vi "Handle Incoming Packets.vi"(8 "error in (no error)":errorcluster, 9 "SessionMailbox":refnum<queue>, 10 "Incoming Packet":refnum<class "ControlPacket.lvclass">, 11 "Server in":refnum<class "Server.lvclass">) -> (0 "error out":errorcluster, 1 "SessionMailbox out":refnum<queue>, 2 "Outgoing":T1, 3 "Server out":refnum<class "Server.lvclass">)   [LabVIEW 2013, in "MQTT Server.lvlib" / "Server.lvclass"]
uses:
  Server.lvclass
  <vilib>/LabVIEW Open Source Project/MQTT Control Packets/Control Packets/ControlPacket/ControlPacket.lvclass
  <vilib>/LabVIEW Open Source Project/MQTT Connection/MQTT_Base/Base Class/Response -- cluster.ctl
  Server.lvclass/Server.ctl
  PacketTracer/PacketTracer.lvclass
  <vilib>/LabVIEW Open Source Project/MQTT Connection/MQTT_Base/Base Class/MQTT_Base.lvclass
  <vilib>/LabVIEW Open Source Project/MQTT Control Packets/Control Packets/CONNECT/CONNECT.lvclass
  <vilib>/LabVIEW Open Source Project/MQTT Control Packets/Control Packets/CONNACK/Connect Return Code -- enum.ctl
  <vilib>/LabVIEW Open Source Project/MQTT Control Packets/Control Packets/DISCONNECT/DISCONNECT.lvclass
  <vilib>/LabVIEW Open Source Project/MQTT Control Packets/Control Packets/PUBLISH/PUBLISH.lvclass
  <vilib>/LabVIEW Open Source Project/MQTT Connection/MQTT_Base/Base Class/MQTT_Base.lvclass/MQTT_Base.ctl
  <vilib>/LabVIEW Open Source Project/MQTT Control Packets/Control Packets/ControlPacket/ControlPacket.lvclass/ControlPacket.ctl
  <vilib>/LabVIEW Open Source Project/MQTT Control Packets/Control Packets/Ack/Ack.lvclass
  <vilib>/LabVIEW Open Source Project/MQTT Control Packets/Control Packets/PUBREL/PUBREL.lvclass
  <vilib>/LabVIEW Open Source Project/MQTT Control Packets/Control Packets/SUBSCRIBE/SUBSCRIBE.lvclass
  <vilib>/LabVIEW Open Source Project/MQTT Control Packets/Control Packets/SUBACK/Subscription Success Code.ctl
  <vilib>/LabVIEW Open Source Project/MQTT Control Packets/Control Packets/ControlPacket/QualityOfService -- enum.ctl
  <vilib>/LabVIEW Open Source Project/MQTT Control Packets/Control Packets/UNSUBSCRIBE/UNSUBSCRIBE.lvclass
  <vilib>/LabVIEW Open Source Project/MQTT Control Packets/Control Packets/PINGREQ/PINGREQ.lvclass
  PacketCollection/PacketCollection.lvclass/PacketCollection.ctl
  <vilib>/LabVIEW Open Source Project/MQTT Control Packets/Control Packets/PUBREC/PUBREC.lvclass
  <vilib>/LabVIEW Open Source Project/MQTT Control Packets/Control Packets/CONNACK/CONNACK.lvclass
  <vilib>/LabVIEW Open Source Project/MQTT Control Packets/Control Packets/SUBACK/SUBACK.lvclass
  PacketCollection/PacketCollection.lvclass
  <vilib>/LabVIEW Open Source Project/MQTT Control Packets/Control Packets/PINGRESP/PINGRESP.lvclass
  <vilib>/LabVIEW Open Source Project/MQTT Control Packets/Control Packets/UNSUBACK/UNSUBACK.lvclass
  StoredSessions/StoredSessions.lvclass
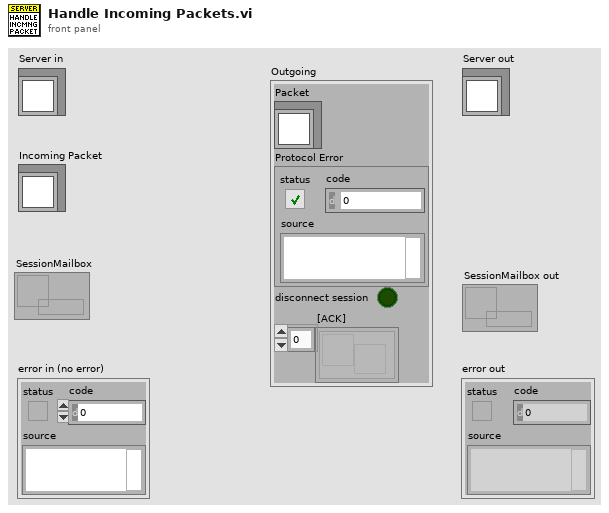
[diagram p1: front panel]
types:
  T1 = typedef "MQTT Base.lvlib/MQTT_Base.lvclass/Response -- cluster.ctl" = cluster{"Packet":refnum<class "ControlPacket.lvclass">, "Protocol Error":errorcluster, "disconnect session":bool, "[ACK]":refnum<notifier>[]}
  T2 = typedef "MQTT_Control_Packets.lvlib/CONNACK.lvclass/Connect Return Code -- enum.ctl" = enum16{"Connection accepted", "Unacceptable protocol version", "Identifier Rejected", "Server Unavailable", "Bad Username or Password", "Not Authorized"}
  T3 = typedef "MQTT_Control_Packets.lvlib/SUBACK.lvclass/Subscription Success Code.ctl" = cluster{"Subscription Failure":bool, "QoS":T4}
  T4 = typedef "MQTT_Control_Packets.lvlib/ControlPacket.lvclass/QualityOfService -- enum.ctl" = enum16{"0 (At Most Once)", "1 (At Least Once)", "2 (Exactly Once)"}
  T5 = typedef "MQTT_Control_Packets.lvlib/ControlPacket.lvclass/Control Packet Type -- enum.ctl" = enum16{"Reserved", "CONNECT", "CONNACK", "PUBLISH", "PUBACK", "PUBREC", "PUBREL", "PUBCOMP", "SUBSCRIBE", "SUBACK", "UNSUBSCRIBE", "UNSUBACK", "PINGREQ", "PINGRESP", "DISCONNECT", "AUTH"}
  T6 = typedef "MQTT_Control_Packets.lvlib/CONNECT.lvclass/ConnectPayload -- cluster.ctl" = cluster{"Will Topic":string, "Will Message":string, "Username":string, "Password":string}
  T7 = typedef "MQTT_Control_Packets.lvlib/CONNECT.lvclass/ConnectFlags -- cluster.ctl" = cluster{"Reserved":bool, "Clean Session":bool, "Will Flag":bool, "Will QoS 1":bool, "Will QoS 2":bool, "Will Retain":bool, "Password Flag":bool, "User Name Flag":bool}
  T8 = typedef "MQTT Server.lvlib/StoredSessions.lvclass/Session State -- cluster.ctl" = cluster{"Client ID":string, "Subscriptions":T9[], "PUBREC":u16[]}
  T9 = typedef "MQTT_Control_Packets.lvlib/SUBSCRIBE.lvclass/Topic Subscription -- cluster.ctl" = cluster{"Topic Filter":string, "QoS":T4}
  T10 = typedef "MQTT Base.lvlib/MQTT_Base.lvclass/Public Events -- cluster.ctl" = cluster{"Stop Event":refnum<user-event>, "Error Event":refnum<user-event>, "Inbound Message":refnum<user-event>}
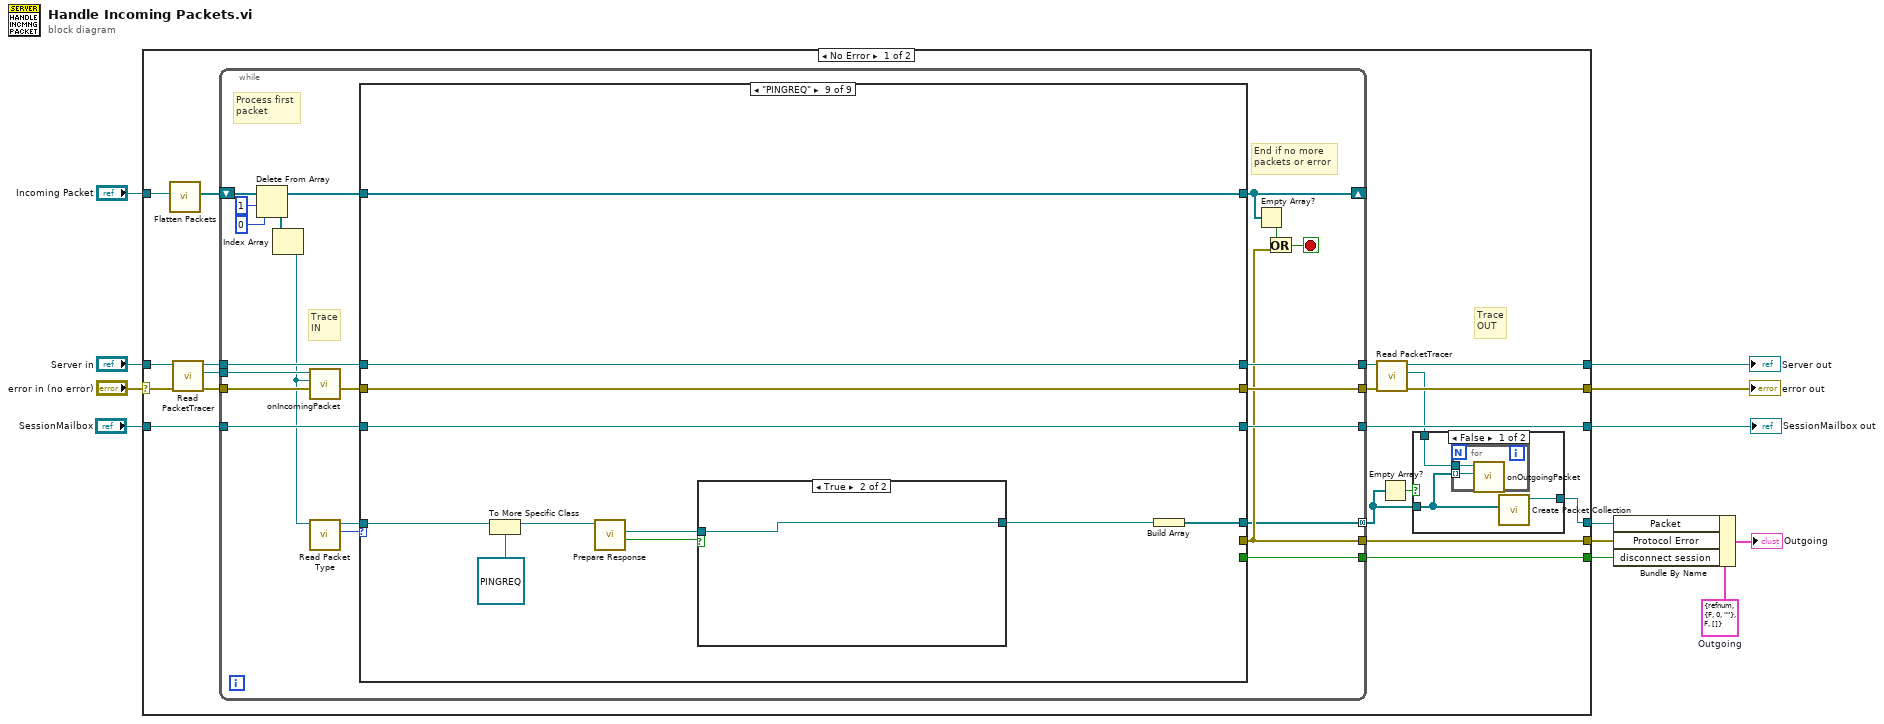
[diagram p0: block diagram]
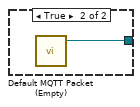
[diagram p2: hidden frame]
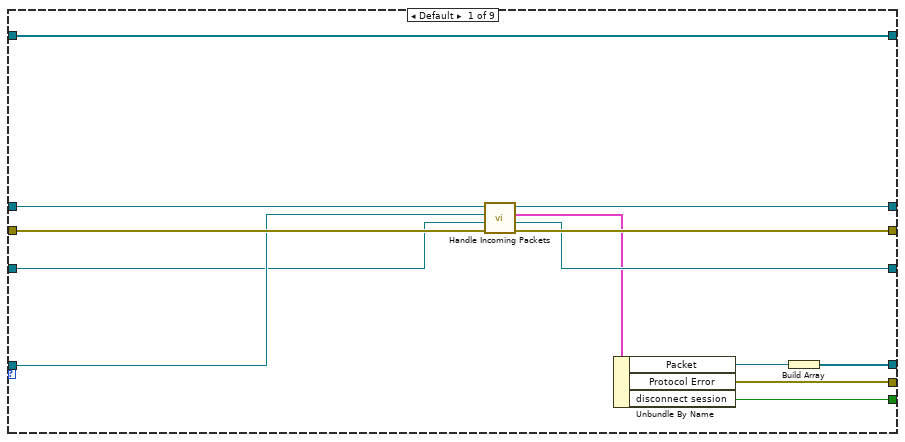
[diagram p3: hidden frame]
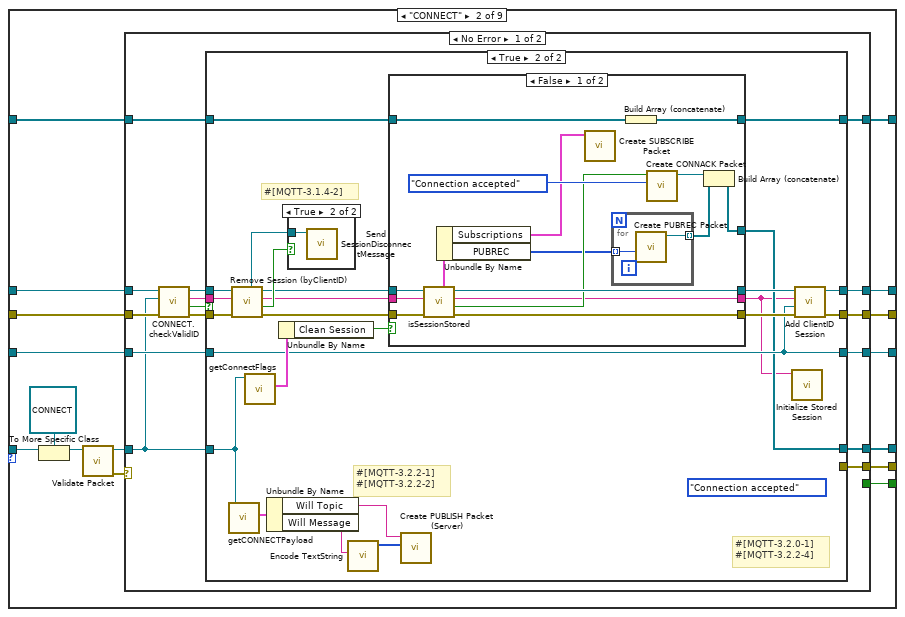
[diagram p4: hidden frame]
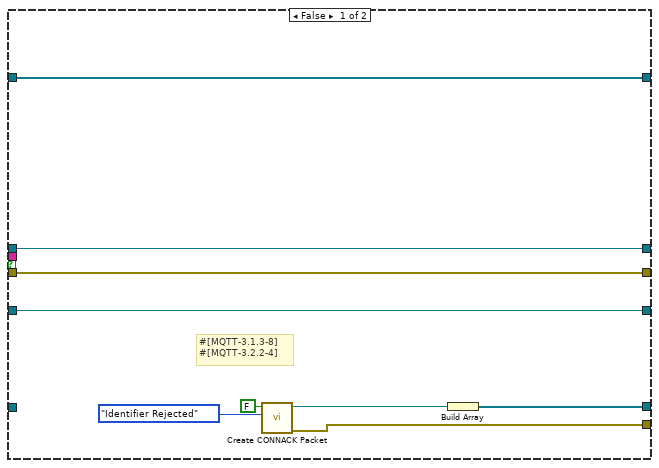
[diagram p5: hidden frame]
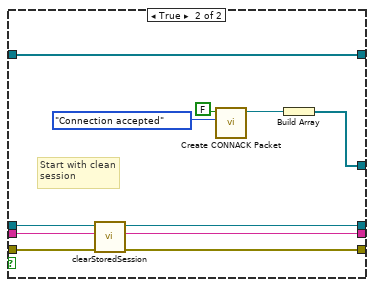
[diagram p6: hidden frame]
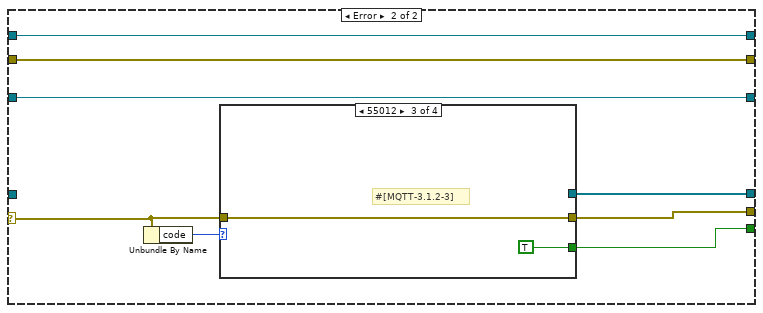
[diagram p8: hidden frame]
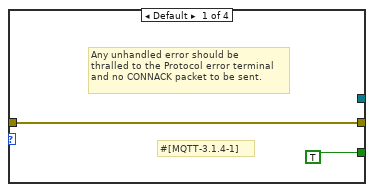
[diagram p9: hidden frame]
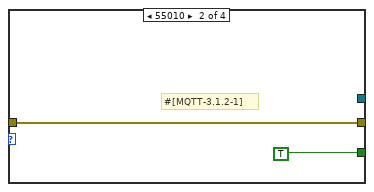
[diagram p10: hidden frame]
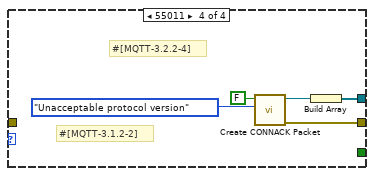
[diagram p11: hidden frame]
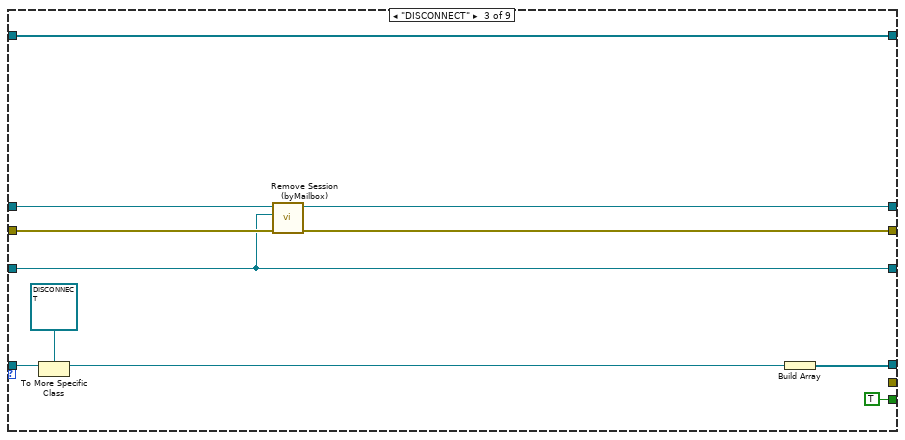
[diagram p12: hidden frame]
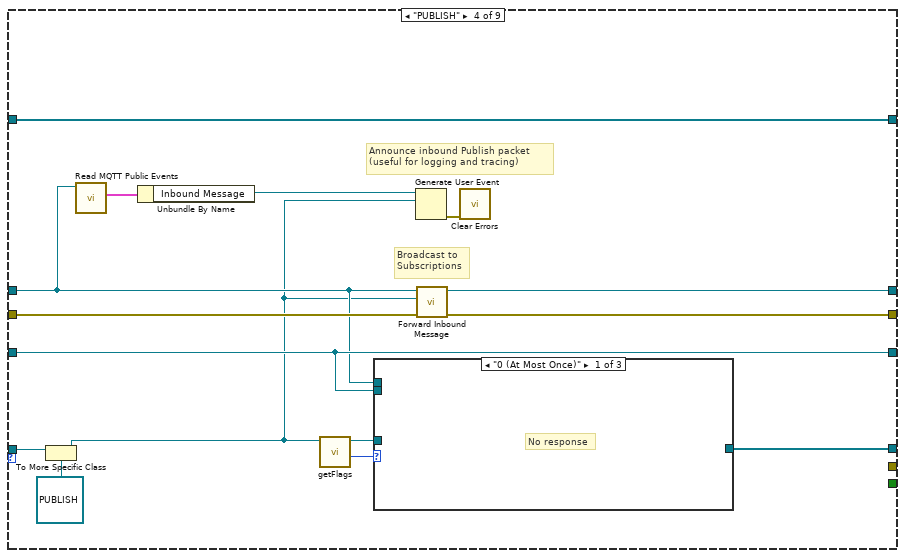
[diagram p13: hidden frame]
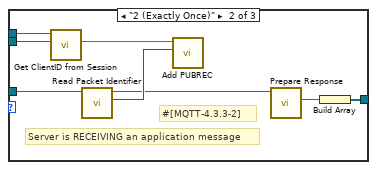
[diagram p14: hidden frame]
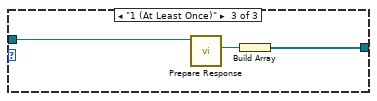
[diagram p15: hidden frame]
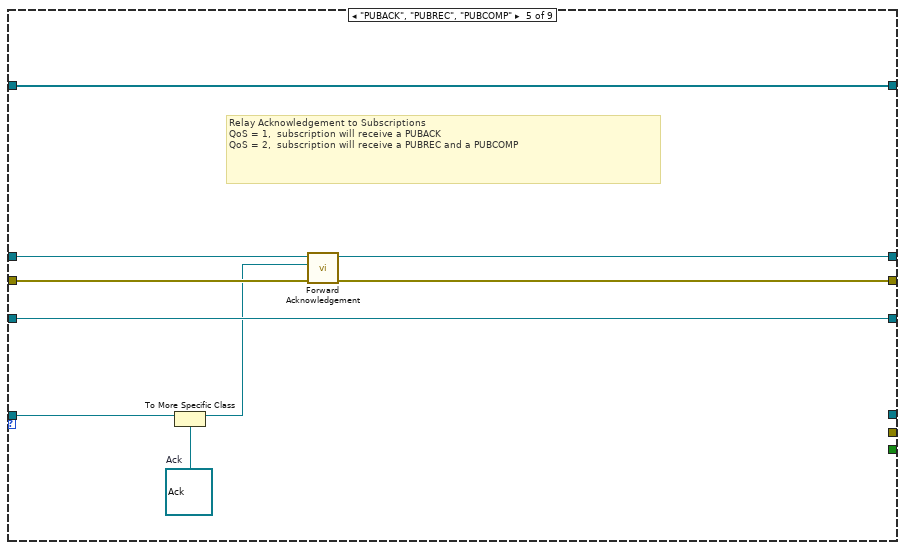
[diagram p16: hidden frame]
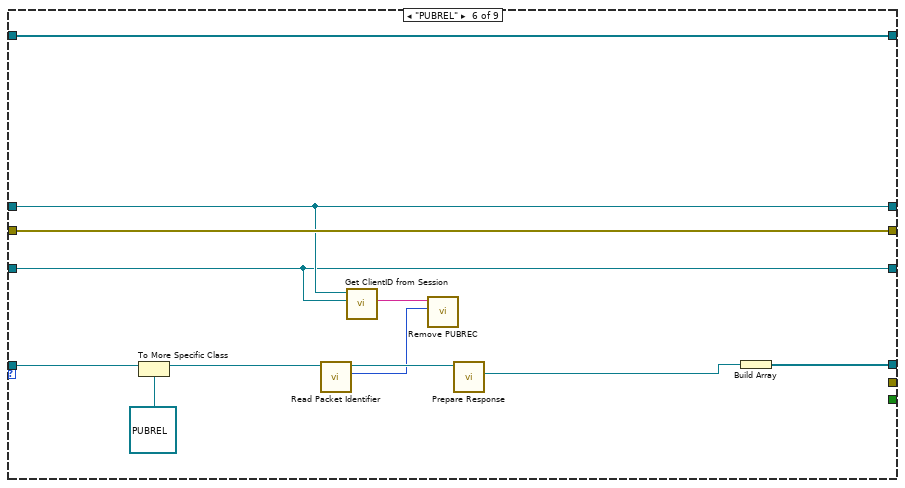
[diagram p17: hidden frame]
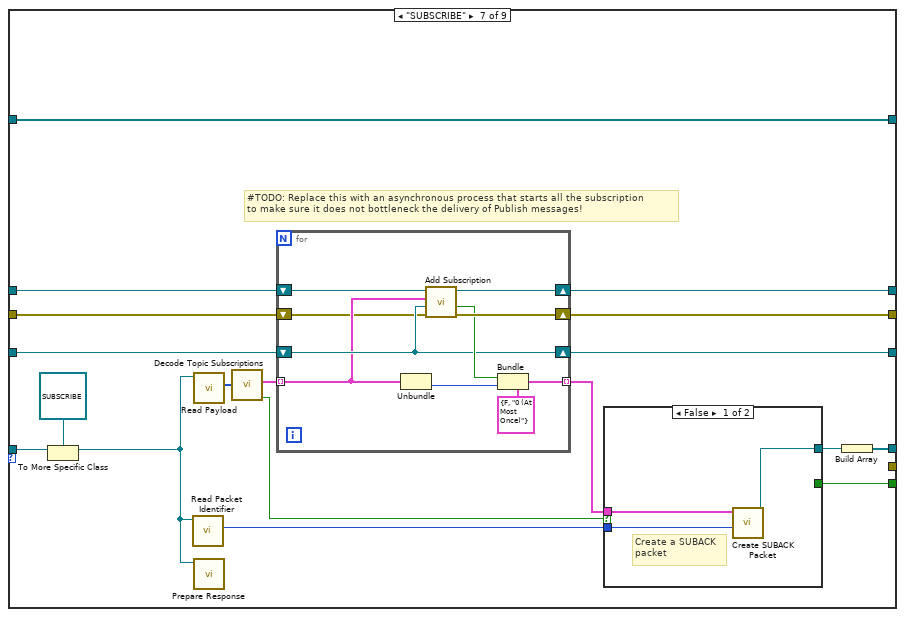
[diagram p18: hidden frame]
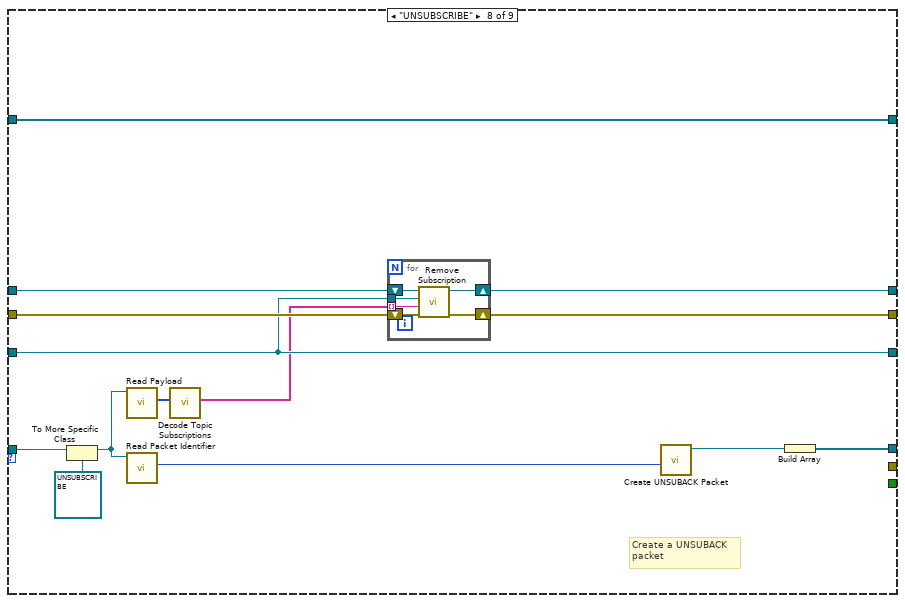
[diagram p20: hidden frame]
diagram:
  w7 = T1 {"Packet"=refnum, "Protocol Error"={"status"=FALSE, "code"=0, "source"=""}, "disconnect session"=FALSE, "[ACK]"=[]}  # Outgoing
  n1 = case shown="No Error" "error in (no error)" {
    selector: "error in (no error)" -> [w22 w310]
    tunnel: [w15 w310] -> w11
    tunnel: [w17 w309] -> w9
    tunnel: "Server in" -> [w20 w309]
    tunnel: "Incoming Packet" -> [w27 _]
    tunnel: [w23 _] -> w6
    tunnel: [w31 _] -> w2
    tunnel: "SessionMailbox" -> [w30 w308]
    tunnel: [w29 w308] -> w1
    tunnel: [w28 _] -> w4
    frame No Error {
      # "Trace\nOUT"
      n2 = call "Flatten Packets.vi"("Incoming Packet"=w27) -> ("Packets"=w26:refnum<class "ControlPacket.lvclass">[])  [unwired: 10 in]
      n3 = call "Read PacketTracer.vi"("error in (no error)"=w22, "Server in"=w20) -> ("error out"=w21:errorcluster, "PacketTracer"=w18:refnum<class "PacketTracer.lvclass">, "Server out"=w19:refnum<class "Server.lvclass">)  [unwired: 7 in]
      n4 = while {
        tunnel: w21 -> [w56]
        tunnel: w19 -> [w40]
        tunnel: [w55] -> w16
        tunnel: [w54] -> w14
        tunnel: [w41] -> w24 mode=concatenating
        tunnel: [w44] -> w31
        tunnel: w30 -> [w53]
        tunnel: [w52] -> w29
        tunnel: [w51] -> w28
        shift-right: [w48] -> _
        shift-left: w26 -> [w50]
        tunnel: w18 -> [w39]
        stop <- w42 stop-if-true
        # "Trace\nIN"
        # "End if no more\npackets or error"
        # "Process first\npacket"
        n5 = Delete From Array(array=w50, length=1, index=0) -> (deleted portion=w45:refnum<class "ControlPacket.lvclass">[], array with subset deleted=w49:refnum<class "ControlPacket.lvclass">[])
        n6 = Index Array(array=w45) -> (element=w38:refnum<class "ControlPacket.lvclass">)  [unwired: 1 in]
        n7 = call-dynamic "onIncomingPacket.vi"("ControlPacket"=w38, "PacketTracer in"=w39) -> ()  [unwired: 10 in]
        n8 = call <vilib>:"Read Packet Type.vi"("ControlPacket in"=w38) -> ("Control Packet Type"=w58:T5, "ControlPacket out"=w57:refnum<class "ControlPacket.lvclass">)  [unwired: 9 in]
        n9 = case shown="\"PINGREQ\"" w58 {
          tunnel: w57 -> [w67 w84 w195 w210 w229 w241 w260 w288 w302]
          tunnel: w56 -> [w69 w81 w191 w208 w228 w242 w248 w284 w304]
          tunnel: w40 -> [w71 w82 w193 w199 w226 w236 w247 w282 w305]
          tunnel: [w70 w79 w192 w207 w225 w236 w254 w281 w305] -> w55
          tunnel: [w68 w80 w190 w206 w227 w242 w253 w283 w304] -> w54
          tunnel: w53 -> [w66 w78 w189 w203 w230 w235 w246 w280 w303]
          tunnel: [w59 w77 w185 w201 _ w237 w244 w275 w297] -> w41
          tunnel: [w63 w76 _ _ _ _ _ _ _] -> w44
          tunnel: [w65 w75 w189 w203 w230 w235 w252 w280 w303] -> w52
          tunnel: [w62 w72 TRUE ("disconnect session") _ _ _ w250 _ _] -> w51
          tunnel: [w61 w73 w186 w205 w222 w239 w245 w277 w299] -> w48
          tunnel: w49 -> [w61 w74 w186 w205 w222 w239 w245 w277 w299]
          frame Default {
            n10 = call-parent "Handle Incoming Packets.vi"("error in (no error)"=w69, "SessionMailbox"=w66, "Incoming Packet"=w67, "MQTT_Base in"=w71) -> ("error out"=w68:errorcluster, "SessionMailbox out"=w65:refnum<queue>, "Outgoing"=w64:T1, "MQTT_Base out"=w70:refnum<class "Server.lvclass">)  [unwired: 4 in]
            n11 = Unbundle By Name(w64) -> ("Packet"=w60:refnum<class "ControlPacket.lvclass">, "Protocol Error"=w63:errorcluster, "disconnect session"=w62:bool)
            n12 = Build Array(w60) -> (w59:refnum<class "ControlPacket.lvclass">[])
          }
          frame "CONNECT" {
            n13 = To More Specific Class(target class=refnum<class "CONNECT.lvclass"> refnum ("CONNECT.lvclass"), reference=w84) -> (specific class reference=w83:refnum<class "CONNECT.lvclass">)  [unwired: 1 in, 1 out]
            n14 = call <vilib>:"Validate Packet.vi"("ControlPacket in"=w83) -> ("error out"=w87:errorcluster, "ControlPacket out"=w86:refnum<class "CONNECT.lvclass">)  [unwired: 9 in]
            n15 = case shown="No Error" w87 {
              selector: w87 -> [_ w172]
              tunnel: w86 -> [w91 _]
              tunnel: w82 -> [w96 w171]
              tunnel: w81 -> [w94 w170]
              tunnel: [w101 w170] -> w80
              tunnel: [w102 w171] -> w79
              tunnel: w78 -> [w100 w167]
              tunnel: [w99 w169] -> w77
              tunnel: [w98 w168] -> w76
              tunnel: [w97 w167] -> w75
              tunnel: w74 -> [w89 _]
              tunnel: [w88 _] -> w73
              tunnel: [_ w166] -> w72
              frame No Error {
                n16 = call "CONNECT.checkValidID.vi"("error in (no error)"=w94, "CONNECT"=w91, "Server in"=w96) -> ("error out"=w93:errorcluster, "valid ID"=w90:bool, "client ID"=w92:string, "Server out"=w95:refnum<class "Server.lvclass">)  [unwired: 5 in]
                n17 = case shown="True" w90 {
                  tunnel: [w106 w128] -> w102
                  tunnel: [w107 w129] -> w101
                  tunnel: w100 -> [w108 w116]
                  tunnel: [w103 w115] -> w99
                  tunnel: [w109 _] -> w98
                  tunnel: [w108 w116] -> w97
                  tunnel: w95 -> [w106 w125]
                  tunnel: w93 -> [w107 w126]
                  tunnel: w92 -> [_ w127]
                  tunnel: w91 -> [_ w135]
                  tunnel: w89 -> [w105 w113]
                  tunnel: [w105 w112] -> w88
                  frame False {
                    # "#[MQTT-3.1.3-8]\n#[MQTT-3.2.2-4]"
                    n18 = call <vilib>:"Create CONNACK Packet.vi"("Return Code"=Connect_Return_Code_--_enum."Identifier Rejected", "Session Present"=FALSE) -> ("error out"=w109:errorcluster, "CONNACK"=w104:refnum<class "CONNACK.lvclass">)  [unwired: 7 in, 1 out]
                    n19 = Build Array(w104) -> (w103:refnum<class "CONNACK.lvclass">[])
                  }
                  frame True {
                    (unwired) Connect_Return_Code_--_enum."Connection accepted" ("Return Code")
                    # "#[MQTT-3.1.4-2]"
                    # "#[MQTT-3.2.2-1]\n#[MQTT-3.2.2-2]"
                    # "#[MQTT-3.2.0-1]\n#[MQTT-3.2.2-4]"
                    n20 = call <vilib>:"getCONNECTPayload.vi"("CONNECT in"=w135) -> ("Payload"=w134:T6)  [unwired: 9 in, 1 out]
                    n21 = call "Remove Session (byClientID).vi"("error in (no error)"=w126, "Client ID"=w127, "MQTT Server"=w125) -> ("error out"=w120:errorcluster, "removed"=w123:bool, "Client ID dup"=w121:string, "MQTT Server"=w122:refnum<class "Server.lvclass">, "SessionMailbox"=w124:refnum<queue>)  [unwired: 4 in]
                    n22 = call <vilib>:"getConnectFlags.vi"("CONNECT in"=w135) -> ("Connect Flags"=w130:T7)  [unwired: 9 in, 1 out]
                    n23 = Unbundle By Name(w134) -> ("Will Topic"=w133:string, "Will Message"=w131:string)
                    n24 = Unbundle By Name(w130) -> ("Clean Session"=w119:bool)
                    n25 = case shown="True" w123 {
                      tunnel: w124 -> [_ w165]
                      frame False {
                      }
                      frame True {
                        n26 = call "Send SessionDisconnectMessage.vi"("SessionMailbox"=w165) -> ()  [unwired: 10 in, 1 out]
                      }
                    }
                    n27 = call <vilib>:"Encode TextString.vi"("Text String"=w131) -> ("Length-Prefixed Field"=w132:u8[])  [unwired: 10 in]
                    n28 = case shown="False" w119 {
                      tunnel: w122 -> [w151 w164]
                      tunnel: w121 -> [w147 w163]
                      tunnel: w120 -> [w150 w162]
                      tunnel: [w149 w161] -> w118
                      tunnel: [w148 w160] -> w117
                      tunnel: [w143 w157] -> w114
                      tunnel: [w137 w154] -> w115
                      tunnel: w113 -> [w142 w156]
                      tunnel: [w141 w156] -> w112
                      frame False {
                        n29 = call "isSessionStored.vi"("error in"=w150, "Client ID"=w147, "MQTT Server"=w151) -> ("error out"=w149:errorcluster, "Session Present"=w145:bool, "Client ID dup"=w143:string, "MQTT Server out"=w148:refnum<class "Server.lvclass">, "Stored Session"=w140:T8)  [unwired: 4 in]
                        n30 = Unbundle By Name(w140) -> ("Subscriptions"=w136:T9[], "PUBREC"=w139:u16[])
                        n31 = call <vilib>:"Create SUBSCRIBE Packet.vi"("Topic Subscriptions"=w136) -> ()  [unwired: 8 in, 3 out]
                        n32 = for {
                          tunnel: w139 -> [w153] mode=indexing
                          tunnel: [w152] -> w138 mode=indexing
                          n33 = call <vilib>:"Create PUBREC Packet.vi"("Packet ID"=w153) -> ("PUBREC out"=w152:refnum<class "PUBREC.lvclass">)  [unwired: 8 in, 2 out]
                        }
                        n34 = Build Array (concatenate)(w142) -> (w141:refnum<class "ControlPacket.lvclass">[])
                        n35 = call <vilib>:"Create CONNACK Packet.vi"("Return Code"=Connect_Return_Code_--_enum."Connection accepted", "Session Present"=w145) -> ("CONNACK"=w144:refnum<class "CONNACK.lvclass">)  [unwired: 7 in, 2 out]
                        n36 = Build Array (concatenate)(w144, w138) -> (w137:refnum<class "Ack.lvclass">[])
                      }
                      frame True {
                        # "Start with clean session"
                        n37 = call "clearStoredSession.vi"("error in"=w162, "Client ID"=w163, "MQTT Server"=w164) -> ("error out"=w161:errorcluster, "Client ID dup"=w157:string, "MQTT Server out"=w160:refnum<class "Server.lvclass">)  [unwired: 5 in, 1 out]
                        n38 = call <vilib>:"Create CONNACK Packet.vi"("Return Code"=Connect_Return_Code_--_enum."Connection accepted", "Session Present"=FALSE) -> ("CONNACK"=w155:refnum<class "CONNACK.lvclass">)  [unwired: 7 in, 2 out]
                        n39 = Build Array(w155) -> (w154:refnum<class "CONNACK.lvclass">[])
                      }
                    }
                    n40 = call <vilib>:"Create PUBLISH Packet (Server).vi"("Payload"=w132, "Topic Name"=w133) -> ()  [unwired: 6 in, 4 out]
                    n41 = call "Initialize Stored Session.vi"("Client ID"=w114) -> ()  [unwired: 10 in, 1 out]
                    n42 = call "Add ClientID Session.vi"("error in (no error)"=w118, "SessionMailbox"=w116, "Client ID"=w114, "MQTT Server"=w117) -> ("error out"=w129:errorcluster, "MQTT Server"=w128:refnum<class "Server.lvclass">)  [unwired: 6 in]
                  }
                }
              }
              frame Error {
                n43 = Unbundle By Name(w172) -> ("code"=w173:i32)
                n44 = case shown="55012" w173 {
                  tunnel: [_ _ _ w180] -> w169
                  tunnel: [w175 w177 w179 w182] -> w168
                  tunnel: w172 -> [w175 w177 w179 _]
                  tunnel: [TRUE TRUE TRUE _] -> w166
                  frame Default {
                    # "#[MQTT-3.1.4-1]"
                    # "Any unhandled error should be\nthralled to the Protocol error terminal\nand no CONNACK packet to be sent."
                  }
                  frame 55010 {
                    # "#[MQTT-3.1.2-1]"
                  }
                  frame 55012 {
                    # "#[MQTT-3.1.2-3]"
                  }
                  frame 55011 {
                    # "#[MQTT-3.2.2-4]"
                    # "#[MQTT-3.1.2-2]"
                    n45 = call <vilib>:"Create CONNACK Packet.vi"("Return Code"=Connect_Return_Code_--_enum."Unacceptable protocol version", "Session Present"=FALSE) -> ("error out"=w182:errorcluster, "CONNACK"=w181:refnum<class "CONNACK.lvclass">)  [unwired: 7 in, 1 out]
                    n46 = Build Array(w181) -> (w180:refnum<class "CONNACK.lvclass">[])
                  }
                }
              }
            }
          }
          frame "DISCONNECT" {
            n47 = To More Specific Class(target class=refnum<class "DISCONNECT.lvclass"> refnum ("DISCONNECT.lvclass"), reference=w195) -> (specific class reference=w187:refnum<class "DISCONNECT.lvclass">)  [unwired: 1 in, 1 out]
            n48 = call "Remove Session (byMailbox).vi"("error in (no error)"=w191, "SessionMailbox"=w189, "MQTT Server"=w193) -> ("error out"=w190:errorcluster, "MQTT Server"=w192:refnum<class "Server.lvclass">)  [unwired: 7 in]
            n49 = Build Array(w187) -> (w185:refnum<class "DISCONNECT.lvclass">[])
          }
          frame "PUBLISH" {
            # "Announce inbound Publish packet\n(useful for logging and tracing)"
            # "Broadcast to\nSubscriptions"
            n50 = To More Specific Class(target class=refnum<class "PUBLISH.lvclass"> refnum ("PUBLISH.lvclass"), reference=w210) -> (specific class reference=w197:refnum<class "PUBLISH.lvclass">)  [unwired: 1 in, 1 out]
            n51 = call <vilib>:"Read MQTT Public Events.vi"("MQTT_Base in"=w199) -> ("MQTT Public Events"=w200:T10)  [unwired: 8 in, 2 out]
            n52 = Unbundle By Name(w200) -> ("Inbound Message"=w198:refnum<user-event>)
            n53 = call-dynamic "getFlags.vi"("PUBLISH in"=w197) -> ("QoS"=w204:T4, "PUBLISH out"=w202:refnum<class "PUBLISH.lvclass">)  [unwired: 7 in, 2 out]
            n54 = case shown="\"0 (At Most Once)\"" w204 {
              tunnel: w199 -> [_ w218 _]
              tunnel: w203 -> [_ w217 _]
              tunnel: w202 -> [_ w215 w219]
              tunnel: [_ w211 w220] -> w201
              frame "0 (At Most Once)" {
                # "No response"
              }
              frame "2 (Exactly Once)" {
                # "#[MQTT-4.3.3-2]"
                # "Server is RECEIVING an application message"
                n55 = call "Get ClientID from Session.vi"("SessionMailbox"=w217, "MQTT Server"=w218) -> ("Client ID"=w216:string)  [unwired: 6 in, 3 out]
                n56 = call <vilib>:"Read Packet Identifier.vi"("ControlPacket in"=w215) -> ("Packet Identifier"=w214:u16, "ControlPacket out"=w212:refnum<class "PUBLISH.lvclass">)  [unwired: 8 in, 1 out]
                n57 = call "Add PUBREC.vi"("Packet Identifier"=w214, "Client ID"=w216) -> ()  [unwired: 9 in, 1 out]
                n58 = call-dynamic "Prepare Response.vi"("PUBLISH in"=w212) -> ("ControlPacket response"=w213:refnum<class "ControlPacket.lvclass">)  [unwired: 7 in, 3 out]
                n59 = Build Array(w213) -> (w211:refnum<class "ControlPacket.lvclass">[])
              }
              frame "1 (At Least Once)" {
                n60 = call-dynamic "Prepare Response.vi"("PUBLISH in"=w219) -> ("ControlPacket response"=w221:refnum<class "ControlPacket.lvclass">)  [unwired: 7 in, 3 out]
                n61 = Build Array(w221) -> (w220:refnum<class "ControlPacket.lvclass">[])
              }
            }
            n62 = Generate User Event(user event=w198, event data cluster=w197) -> (error out=w196:errorcluster)  [unwired: 2 in, 1 out]
            n63 = call "Forward Inbound Message.vi"("error in (no error)"=w208, "Inbound Message"=w197, "MQTT Server"=w199) -> ("error out"=w206:errorcluster, "MQTT Server"=w207:refnum<class "Server.lvclass">)  [unwired: 7 in]
            n64 = call <vilib>:"Clear Errors.vi"("error in (no error)"=w196) -> ()  [unwired: 6 in, 1 out]
          }
          frame "PUBACK", "PUBREC", "PUBCOMP" {
            w224 = refnum<class "Ack.lvclass"> refnum  # Ack
            # "Relay Acknowledgement to Subscriptions\nQoS = 1,  subscription will receive a PUBACK\nQoS = 2,  subscription will receive a PUBREC and a PUBCOMP"
            n65 = To More Specific Class(target class=w224, reference=w229) -> (specific class reference=w223:refnum<class "Ack.lvclass">)  [unwired: 1 in, 1 out]
            n66 = call "Forward Acknowledgement.vi"("error in (no error)"=w228, "Acknowledgement"=w223, "MQTT Server"=w226) -> ("error out"=w227:errorcluster, "MQTT Server"=w225:refnum<class "Server.lvclass">)  [unwired: 7 in]
          }
          frame "PUBREL" {
            n67 = To More Specific Class(target class=refnum<class "PUBREL.lvclass"> refnum ("PUBREL.lvclass"), reference=w241) -> (specific class reference=w233:refnum<class "PUBREL.lvclass">)  [unwired: 1 in, 1 out]
            n68 = call <vilib>:"Read Packet Identifier.vi"("ControlPacket in"=w233) -> ("Packet Identifier"=w231:u16, "ControlPacket out"=w232:refnum<class "PUBREL.lvclass">)  [unwired: 8 in, 1 out]
            n69 = call "Get ClientID from Session.vi"("SessionMailbox"=w235, "MQTT Server"=w236) -> ("Client ID"=w234:string)  [unwired: 6 in, 3 out]
            n70 = call "Remove PUBREC.vi"("Packet Identifier"=w231, "Client ID"=w234) -> ()  [unwired: 9 in, 1 out]
            n71 = call-dynamic "Prepare Response.vi"("PUBREL in"=w232) -> ("ControlPacket response"=w238:refnum<class "ControlPacket.lvclass">)  [unwired: 7 in, 3 out]
            n72 = Build Array(w238) -> (w237:refnum<class "ControlPacket.lvclass">[])
          }
          frame "SUBSCRIBE" {
            # "#TODO: Replace this with an asynchronous process that starts all the subscription\nto make sure it does not bottleneck the delivery of Publish messages!"
            n73 = To More Specific Class(target class=refnum<class "SUBSCRIBE.lvclass"> refnum ("SUBSCRIBE.lvclass"), reference=w260) -> (specific class reference=w249:refnum<class "SUBSCRIBE.lvclass">)  [unwired: 1 in, 1 out]
            n74 = call <vilib>:"Read Packet Identifier.vi"("ControlPacket in"=w249) -> ("Packet Identifier"=w257:u16)  [unwired: 8 in, 2 out]
            n75 = call <vilib>:"Read Payload.vi"("ControlPacket in"=w249) -> ("Payload"=w258:u8[])  [unwired: 9 in, 1 out]
            n76 = call-dynamic "Prepare Response.vi"("ControlPacket in"=w249) -> ()  [unwired: 7 in, 4 out]
            n77 = call <vilib>:"Decode Topic Subscriptions.vi"("Payload"=w258) -> ("invalid UTF8"=w251:bool, "Topic Subscriptions"=w256:T9[])  [unwired: 8 in, 1 out]
            n78 = for {
              tunnel: w256 -> [w267] mode=indexing
              tunnel: [w274] -> w255 mode=indexing
              shift-right: [w270] -> w254
              shift-left: w247 -> [w266]
              shift-right: [w271] -> w253
              shift-left: w248 -> [w265]
              shift-right: [w268] -> w252
              shift-left: w246 -> [w268]
              n79 = Unbundle(w267) -> ("QoS"=w272:T4)  [unwired: 1 out]
              n80 = call "Add Subscription.vi"("error in (no error)"=w265, "SessionMailbox"=w268, "Topic Subscription"=w267, "MQTT Server"=w266) -> ("error out"=w271:errorcluster, "Failed"=w269:bool, "MQTT Server"=w270:refnum<class "Server.lvclass">)  [unwired: 5 in]
              n81 = Bundle(cluster=T3 {"Subscription Failure"=FALSE, "QoS"=enum."0 (At Most Once)"} ("Topic Subscription"), "Subscription Failure"=w269, "QoS"=w272) -> (w274:T3)
            }
            n82 = case shown="False" w251 {
              selector: w251 -> [_ w264]
              tunnel: w257 -> [w263 _]
              tunnel: w255 -> [w262 _]
              tunnel: [w261 _] -> w243
              tunnel: [_ w264] -> w250
              frame False {
                # "Create a SUBACK\npacket"
                n83 = call <vilib>:"Create SUBACK Packet.vi"("Packet ID"=w263, "Return Codes"=w262) -> ("SUBACK"=w261:refnum<class "SUBACK.lvclass">)  [unwired: 7 in, 2 out]
              }
              frame True {
                # "Invalid UTF8 string"
              }
            }
            n84 = Build Array(w243) -> (w244:refnum<class "SUBACK.lvclass">[])
          }
          frame "UNSUBSCRIBE" {
            # "Create a UNSUBACK\npacket"
            n85 = To More Specific Class(target class=refnum<class "UNSUBSCRIBE.lvclass"> refnum ("UNSUBSCRIBE.lvclass"), reference=w288) -> (specific class reference=w287:refnum<class "UNSUBSCRIBE.lvclass">)  [unwired: 1 in, 1 out]
            n86 = call <vilib>:"Read Payload.vi"("ControlPacket in"=w287) -> ("Payload"=w285:u8[])  [unwired: 9 in, 1 out]
            n87 = call <vilib>:"Read Packet Identifier.vi"("ControlPacket in"=w287) -> ("Packet Identifier"=w278:u16)  [unwired: 8 in, 2 out]
            n88 = call <vilib>:"Decode Topic Subscriptions.vi"("Payload"=w285) -> ("Topic Subscriptions"=w279:string[])  [unwired: 9 in, 1 out]
            n89 = for {
              tunnel: w280 -> [w290]
              shift-right: [w291] -> w281
              shift-left: w282 -> [w292]
              shift-right: [w293] -> w283
              shift-left: w284 -> [w294]
              tunnel: w279 -> [w289] mode=indexing
              n90 = call "Remove Subscription.vi"("error in (no error)"=w294, "Topic Filter"=w289, "SessionMailbox"=w290, "MQTT Server"=w292) -> ("error out"=w293:errorcluster, "MQTT Server"=w291:refnum<class "Server.lvclass">)  [unwired: 5 in, 1 out]
            }
            n91 = call <vilib>:"Create UNSUBACK Packet.vi"("Packet ID"=w278) -> ("UNSUBACK out"=w276:refnum<class "UNSUBACK.lvclass">)  [unwired: 8 in, 2 out]
            n92 = Build Array(w276) -> (w275:refnum<class "UNSUBACK.lvclass">[])
          }
          frame "PINGREQ" {
            n93 = To More Specific Class(target class=refnum<class "PINGREQ.lvclass"> refnum ("PINGREC.lvclass"), reference=w302) -> (specific class reference=w300:refnum<class "PINGREQ.lvclass">)  [unwired: 1 in, 1 out]
            n94 = call-dynamic "Prepare Response.vi"("PINGREQ in"=w300) -> ("response prepared?"=w296:bool, "ControlPacket response"=w295:refnum<class "ControlPacket.lvclass">)  [unwired: 7 in, 2 out]
            n95 = case shown="True" w296 {
              tunnel: [w306 w307] -> w298
              tunnel: w295 -> [_ w307]
              frame False {
                # "Create a PINGRESP\npacket"
                n96 = call <vilib>:"Create PINGRESP Packet.vi"() -> ("PINGRESP out"=w306:refnum<class "PINGRESP.lvclass">)  [unwired: 9 in, 2 out]
              }
              frame True {
              }
            }
            n97 = Build Array(w298) -> (w297:refnum<class "ControlPacket.lvclass">[])
          }
        }
        n98 = Empty Array?(array=w48) -> (empty?=w43:bool)
        n99 = Or(x=w43, y=w44) -> (x .or. y?=w42:bool)
      }
      n100 = call "Read PacketTracer.vi"("error in (no error)"=w14, "Server in"=w16) -> ("error out"=w15:errorcluster, "PacketTracer"=w13:refnum<class "PacketTracer.lvclass">, "Server out"=w17:refnum<class "Server.lvclass">)  [unwired: 7 in]
      n101 = Empty Array?(array=w24) -> (empty?=w25:bool)
      n102 = case shown="False" w25 {
        tunnel: [w34 w37] -> w23
        tunnel: w24 -> [w32 _]
        tunnel: w13 -> [w33 _]
        frame False {
          n103 = for {
            tunnel: w33 -> [w36]
            tunnel: w32 -> [w35] mode=indexing
            n104 = call-dynamic "onOutgoingPacket.vi"("ControlPacket"=w35, "PacketTracer in"=w36) -> ()  [unwired: 10 in]
          }
          n105 = call "Create Packet Collection.vi"("Packets"=w32) -> ("PacketCollection"=w34:refnum<class "PacketCollection.lvclass">)  [unwired: 10 in]
        }
        frame True {
          n106 = call <vilib>:"Default MQTT Packet (Empty).vi"() -> ("No Packet"=w37:refnum<class "ControlPacket.lvclass">)  [unwired: 11 in]
        }
      }
    }
    frame Error {
    }
  }
  "error out" <- w11
  "Server out" <- w9
  "SessionMailbox out" <- w1
  n107 = Bundle By Name(cluster=w7, "Packet"=w6, "Protocol Error"=w2, "disconnect session"=w4) -> (→"Outgoing":T1)
